vi "csb ws build frame.vi"(5 "frame_cap":i32, 6 "frame":u8[](array[numeric]), 7 "mask":u32, 8 "error in (no error)":errorcluster, 9 "opcode":u8, 10 "len":i32, 11 "payload":u8[](array[numeric])) -> (0 "error out":errorcluster, 3 "function return":i32, 4 "frame out":u8[](array[numeric]))   [LabVIEW 2021, in "CANsub_Codec.lvlib"]
doc: "int32_t csb_ws_build_frame(const uint8_t *payload, int32_t len, uint8_t opcode, uint32_t mask,\n uint8_t *frame, int32_t frame_cap);"
uses:
  CANsub_Codec.lvlib
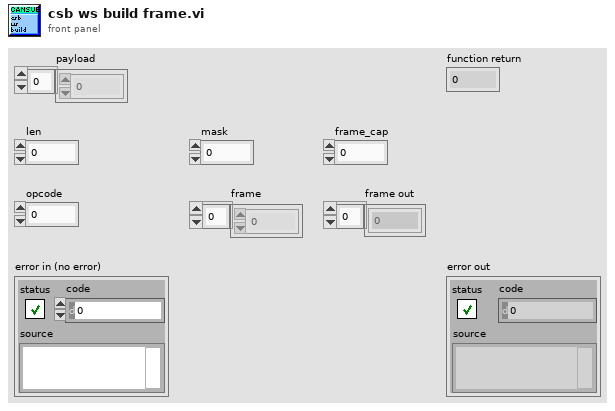
[diagram p1: front panel]
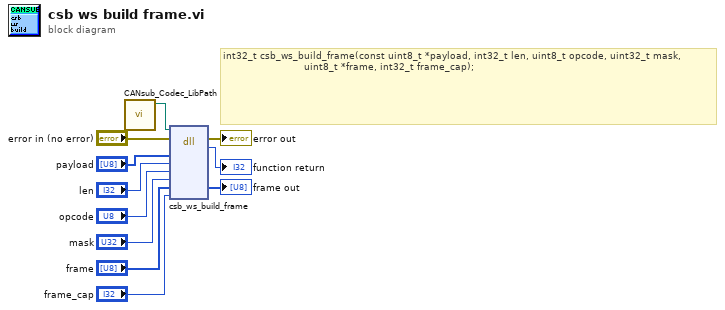
[diagram p0: block diagram]
diagram:
  # "int32_t csb_ws_build_frame(const uint8_t *payload, int32_t len, uint8_t opcode, uint32_t mask,\n                           uint8_t *frame, int32_t frame_cap);"
  n1 = call "CANsub_Codec_LibPath.vi"() -> ("Path"=w1:path)  [unwired: 11 in]
  n2 = dll-call lib="libcansub_codec.*" fn="csb_ws_build_frame"(path in=w1, error in="error in (no error)", "payload"="payload", "len"="len", "opcode"="opcode", "mask"="mask", "frame"="frame", "frame_cap"="frame_cap") -> (error out=→"error out":errorcluster, "return type"=→"function return":i32, "frame"=→"frame out":u8[])  [unwired: 6 in, 1 out]
